vi "Initialization.vi"(8 "error in (no error)":errorcluster, 9 "UI Refs":T1, 10 "user event":T2, 11 "4way Lap in":refnum<class "4way Lap.lvclass">) -> (0 "error out":errorcluster, 3 "4way Lap out":refnum<class "4way Lap.lvclass">)   [LabVIEW 2025, in "Flow Grind.lvlib" / "4way Lap.lvclass"]
uses:
  4way Lap.lvclass
  Users/Public/Documents/Sandia National Labs/TSS Plugin/CEF.lvlibp/Node/UserEventRef.ctl
  Users/Public/Documents/Sandia National Labs/TSS Plugin/Tests/XY Plotter.lvlibp/XY Plotter configuration/XY Plotter configuration.lvclass
  Users/Public/Documents/Sandia National Labs/TSS Plugin/Tests/XY Plotter.lvlibp/XY Plotter configuration/Read XY Plotter.vi
  Users/Public/Documents/Sandia National Labs/TSS Plugin/Tests/XY Plotter.lvlibp/XY  Plotter/XY Plotter.lvclass
  Users/Public/Documents/Sandia National Labs/TSS Plugin/CEF.lvlibp/serializable configuration/CEF_serializable configuration.lvclass
  Users/Public/Documents/Sandia National Labs/TSS Plugin/CEF.lvlibp/Node/CEF_Node.lvclass
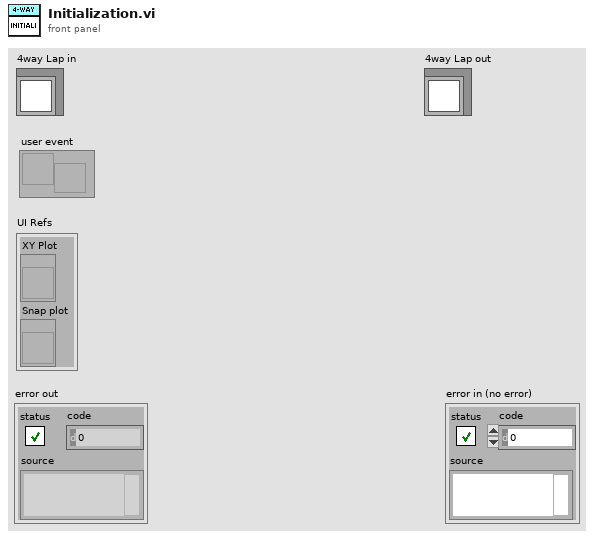
[diagram p1: front panel]
types:
  T1 = cluster{"XY Plot":refnum<vi>, "Snap plot":refnum<vi>}
  T2 = typedef "CEF.lvlibp/CEF_Node.lvclass/UserEventRef.ctl" = refnum<user-event>
  T3 = cluster{"Name":string, "Color":u32, "Style":u8, "Point Style":u8, "Name Visible":bool, "Allow Drag":bool, "Annotation Mode":u32, "Plot":i32, "Index":i32, "Position":cluster{"X":dbl, "Y":dbl}, "X Scale":u32, "Y Scale":u32, "Show Arrow":bool, "Lock Name":bool, "Plot Area":i32, "Label Offset":cluster{"X":dbl, "Y":dbl}}
  T4 = typedef "XY Plotter.lvlibp/XY Plotter configuration.lvclass/XY Plotter.ctl" = cluster{"Data Rate":i32, "Y-Scales":cluster{"Label":string, "Max":dbl, "Min":dbl, "Unit":enum16{"---", "V", "mA", "sec", "dB", "deg", "in/s", "in", "lbf", "Hz", "psi", "gpm"}, "Visible":bool}[], "Note":string, "History Length":i32, "DataLog Path":path, "Plot type":bool, "X-Scales":cluster{"Label":string, "Max":dbl, "Min":dbl, "Unit":enum16{"---", "V", "mA", "sec", "dB", "deg", "in/s", "in", "lbf", "Hz", "psi", "gpm"}, "Visible":bool}[], "Plot List":cluster{"Plot Name":string, "X Scale Index":u32, "Y Scale Index":u32, "Visible":bool}[]}
  T5 = cluster{"Label":string, "Max":dbl, "Min":dbl, "Unit":enum16{"---", "V", "mA", "sec", "dB", "deg", "in/s", "in", "lbf", "Hz", "psi", "gpm"}, "Visible":bool}[]
  T6 = cluster{"Label":string, "Max":dbl, "Min":dbl, "Unit":enum16{"---", "V", "mA", "sec", "dB", "deg", "in/s", "in", "lbf", "Hz", "psi", "gpm"}, "Visible":bool}
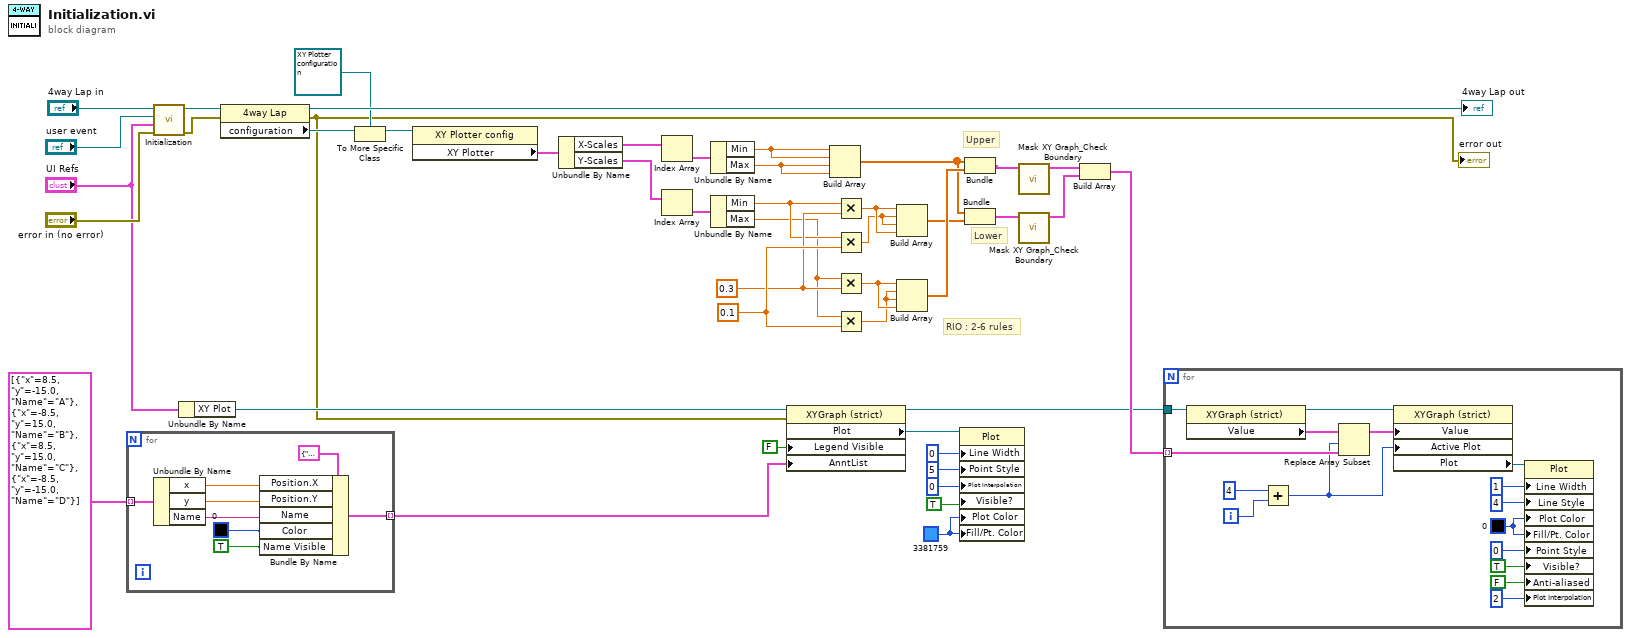
[diagram p0: block diagram]
diagram:
  w4 = u32 3381759 ("Plot Color")
  w19 = 0.1
  w18 = 0.3
  # "RIO : 2-6 rules"
  # "Lower"
  # "Upper"
  n1 = for {
    tunnel: cluster{"x":dbl, "y":dbl, "Name":string}[] [{"x"=8.5, "y"=-15.0, "Name"="A"}, {"x"=-8.5, "y"=15.0, "Name"="B"}, {"x"=8.5, "y"=15.0, "Name"="C"}, {"x"=-8.5, "y"=-15.0, "Name"="D"}] -> [w49] mode=indexing
    tunnel: [w50] -> w1 mode=indexing
    n2 = Unbundle By Name(w49) -> ("x"=w47:dbl, "y"=w46:dbl, "Name"=w48:string)
    n3 = Bundle By Name(cluster=T3 {"Name"="", "Color"=0, "Style"=0, "Point Style"=0, "Name Visible"=FALSE, "Allow Drag"=FALSE, "Annotation Mode"=0, "Plot"=0, "Index"=0, "Position"={"X"=0.0, "Y"=0.0}, "X Scale"=0, "Y Scale"=0, "Show Arrow"=FALSE, "Lock Name"=FALSE, "Plot Area"=0, "Label Offset"={"X"=0.0, "Y"=0.0}}, "Position.X"=w47, "Position.Y"=w46, "Name"=w48, "Color"=u32 0, "Name Visible"=TRUE) -> (w50:T3)
  }
  n4 = call-parent "Initialization.vi"("error in"="error in (no error)", "UI Refs"="UI Refs", "user event"="user event", "XY Plotter"="4way Lap in") -> ("error out"=w30:errorcluster, "XY Plotter out"=w42:refnum<class "4way Lap.lvclass">)  [unwired: 6 in]
  n5 = Unbundle By Name("UI Refs") -> ("XY Plot"=w29:refnum<vi>)
  n6 = property class="4way Lap"(reference=w42, error in=w30) -> (reference out=→"4way Lap out":refnum<class "4way Lap.lvclass">, error out=w15:errorcluster, "configuration"=w39:refnum<class "CEF_serializable configuration.lvclass">)
  "error out" <- w15
  n7 = To More Specific Class(target class=refnum<class "XY Plotter configuration.lvclass"> refnum ("XY Plotter.lvlibp:XY Plotter config"), reference=w39) -> (specific class reference=w38:refnum<class "XY Plotter configuration.lvclass">)  [unwired: 1 in, 1 out]
  n8 = property class="XY Plotter config"(reference=w38) -> ("XY Plotter"=w36:T4)  [unwired: 1 in, 2 out]
  n9 = Unbundle By Name(w36) -> ("X-Scales"=w28:T5, "Y-Scales"=w27:T5)
  n10 = Index Array(array=w28) -> (element=w17:T6)  [unwired: 1 in]
  n11 = Index Array(array=w27) -> (element=w16:T6)  [unwired: 1 in]
  n12 = Unbundle By Name(w17) -> ("Min"=w14:dbl, "Max"=w13:dbl)
  n13 = Unbundle By Name(w16) -> ("Min"=w12:dbl, "Max"=w11:dbl)
  n14 = property class="XYGraph (strict)"(reference=w29, error in=w15, "Legend Visible"=FALSE ("Legend:Visible"), "AnntList"=w1) -> (reference out=w10:refnum<vi>, "Plot"=w6:refnum<vi>)  [unwired: 1 out]
  n15 = Build Array(w14, w14, w13, w13) -> (w23:dbl[])
  n16 = Multiply(x=w12, y=w18) -> (x*y=w22:dbl)
  n17 = Multiply(x=w12, y=w19) -> (x*y=w21:dbl)
  n18 = Multiply(x=w11, y=w18) -> (x*y=w26:dbl)
  n19 = Multiply(x=w11, y=w19) -> (x*y=w25:dbl)
  n20 = Build Array(w22, w21, w21, w22) -> (w20:dbl[])
  n21 = Build Array(w26, w25, w25, w26) -> (w24:dbl[])
  n22 = property class="Plot"(reference=w6, "Line Width"=u8 0, "Point Style"=u8 5, "Plot Interpolation"=u8 0, "Visible?"=TRUE ("Visible"), "Plot Color"=w4, "Fill/Pt. Color"=w4) -> ()  [unwired: 1 in, 2 out]
  n23 = Bundle(w23, w24) -> (w34:cluster{dbl[], dbl[]})  [unwired: 1 in]
  n24 = Bundle(w23, w20) -> (w35:cluster{dbl[], dbl[]})  [unwired: 1 in]
  n25 = call "Mask XY Graph_Check Boundary.vi"("Boundary"=w34) -> ("Closed Boundary"=w32:cluster{"X":dbl[], "Y":dbl[]})  [unwired: 9 in, 1 out]
  n26 = call "Mask XY Graph_Check Boundary.vi"("Boundary"=w35) -> ("Closed Boundary"=w31:cluster{"X":dbl[], "Y":dbl[]})  [unwired: 9 in, 1 out]
  n27 = Build Array(w32, w31) -> (w33:cluster{"X":dbl[], "Y":dbl[]}[])
  n28 = for {
    tunnel: w33 -> [w65] mode=indexing
    tunnel: w10 -> [w66]
    i -> [w64]
    w54 = u32 0 ("Plot Color")
    n29 = property class="XYGraph (strict)"(reference=w66) -> (reference out=w67:refnum<vi>, "Value"=w68:cluster{dbl[], dbl[]}[])  [unwired: 1 in, 1 out]
    n30 = Add(x=4, y=w64) -> (x+y=w62:i32)
    n31 = Replace Array Subset(array=w68, new element=w65, index=w62) -> (w69:cluster{dbl[], dbl[]}[])
    n32 = property class="XYGraph (strict)"(reference=w67, "Value"=w69, "Active Plot"=w62) -> ("Plot"=w55:refnum<vi>)  [unwired: 1 in, 2 out]
    n33 = property class="Plot"(reference=w55, "Line Width"=u8 1, "Line Style"=u8 4, "Plot Color"=w54, "Fill/Pt. Color"=w54, "Point Style"=u8 0, "Visible?"=TRUE ("Visible"), "Anti-aliased"=FALSE, "Plot Interpolation"=u8 2) -> ()  [unwired: 1 in, 2 out]
  }
